vi "FilePaths.vi"(8 "error in":errorcluster) -> (0 "error out":errorcluster, 2 "paths":T1)   [LabVIEW 2014, in "Advanced Configuration Tool.lvlib"]
doc: "This VI has the Path to the Classes and the Glyphs, Additional Behavior might be added if you want to load them from a different path. By default they are in Glyphs folder and Classes folder in the main directory"
uses:
  Advanced Configuration Tool.lvlib
  Controls/FilePaths.ctl
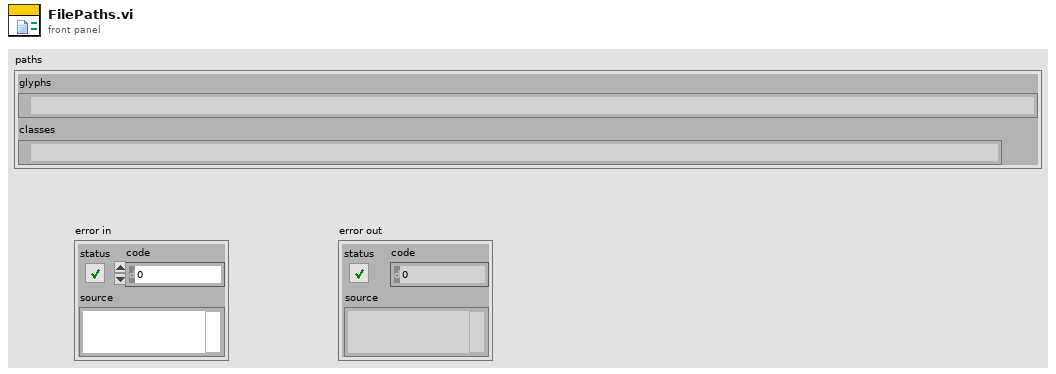
[diagram p1: front panel]
types:
  T1 = typedef "Advanced Configuration Tool.lvlib/FilePaths.ctl" = cluster{"glyphs":path, "classes":path}
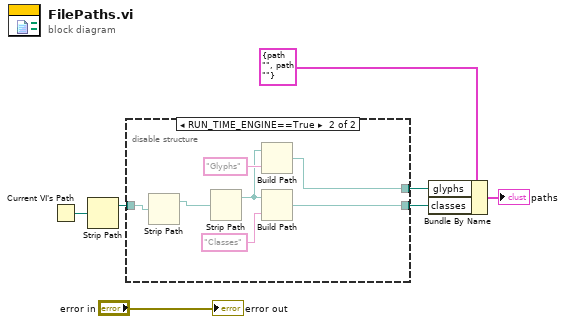
[diagram p0: block diagram]
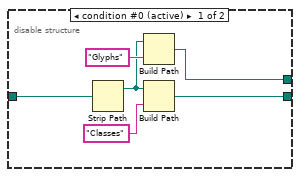
[diagram p2: hidden frame]
diagram:
  n1 = Current VI's Path() -> (path=w2:path)
  n2 = Strip Path(path=w2) -> (stripped path=w1:path)  [unwired: 1 out]
  n3 = disable-structure shown="RUN_TIME_ENGINE==True" {
    disable-tunnel: [w12 w19] -> w5
    disable-tunnel: [w10 w17] -> w3
    disable-tunnel: w1 -> [w8 w15]
    frame condition #0 (active) {
      n4 = Strip Path(path=w8) -> (stripped path=w9:path)  [unwired: 1 out]
      n5 = Build Path(base path=w9, name or relative path="Glyphs") -> (appended path=w12:path)
      n6 = Build Path(base path=w9, name or relative path="Classes") -> (appended path=w10:path)
    }
    frame condition #1 {
      n7 = Strip Path(path=w15) -> (stripped path=w14:path)  [unwired: 1 out]
      n8 = Strip Path(path=w14) -> (stripped path=w16:path)  [unwired: 1 out]
      n9 = Build Path(base path=w16, name or relative path="Glyphs") -> (appended path=w19:path)
      n10 = Build Path(base path=w16, name or relative path="Classes") -> (appended path=w17:path)
    }
  }
  n11 = Bundle By Name(cluster=T1 {"glyphs"=path "", "classes"=path ""} ("Cluster 2"), "glyphs"=w5, "classes"=w3) -> (→"paths":T1)
  "error out" <- "error in"
